vi "check Self Alignment Processing.vi"(8 "error in (no error)":errorcluster, 11 "Keysight 9020A in":refnum<class "Keysight 9020A.lvclass">) -> (0 "error out":errorcluster, 2 "On Alignment Processing":bool, 3 "Keysight 9020A out":refnum<class "Keysight 9020A.lvclass">)   [LabVIEW 2023, in "Spectrum Analyzer.lvlib" / "Keysight 9020A.lvclass"]
uses:
  Keysight 9020A.lvclass
  Keysight 9020A.lvclass/Keysight 9020A.ctl
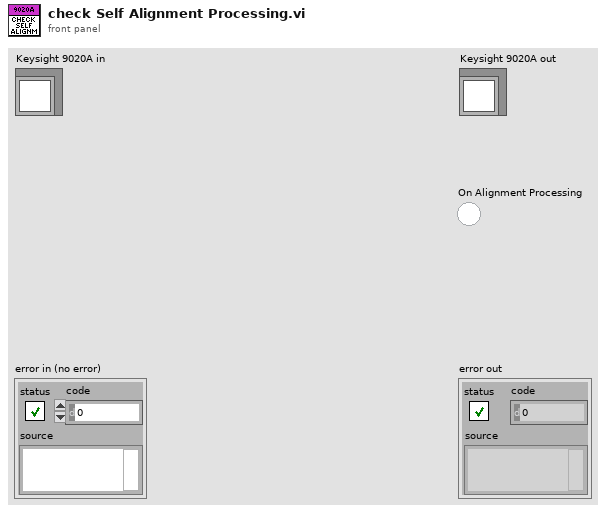
[diagram p1: front panel]
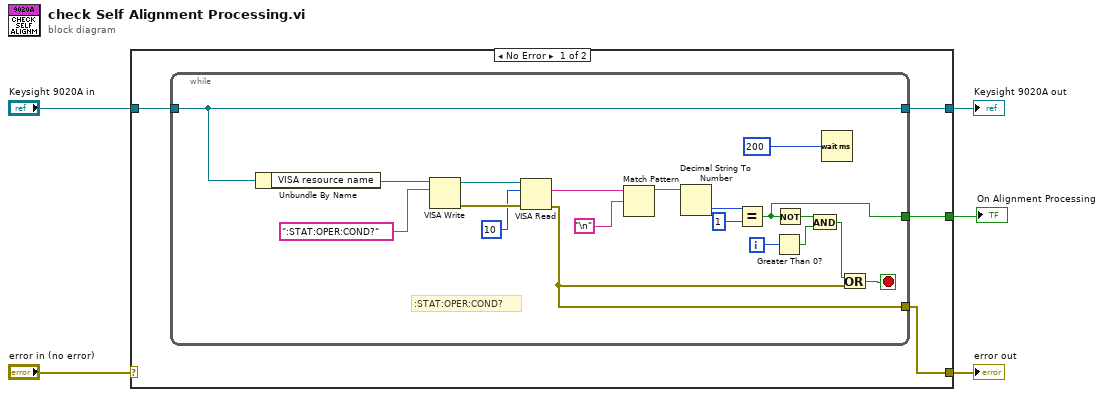
[diagram p0: block diagram]
diagram:
  n1 = case shown="No Error" "error in (no error)" {
    selector: "error in (no error)" -> [_ w30]
    tunnel: [w7 w30] -> w4
    tunnel: [w6 w29] -> w2
    tunnel: "Keysight 9020A in" -> [w9 w29]
    tunnel: [w8 _] -> w1
    frame No Error {
      n2 = while {
        tunnel: w9 -> [w16]
        tunnel: [w11] -> w8
        tunnel: [w17] -> w7
        tunnel: [w16] -> w6
        i -> [w12]
        stop <- w18 stop-if-true
        # ":STAT:OPER:COND?"
        n3 = Unbundle By Name(w16) -> ("VISA resource name"=w28:refnum<visa-resource-name>)
        n4 = VISA Write(VISA resource name=w28, write buffer=":STAT:OPER:COND?") -> (VISA resource name out=w26:refnum<visa-resource-name>, error out=w25:errorcluster)  [unwired: 1 in, 1 out]
        n5 = VISA Read(VISA resource name=w26, byte count=u32 10, error in (no error)=w25) -> (read buffer=w23:string, error out=w17:errorcluster)  [unwired: 2 out]
        n6 = Match Pattern(string=w23, regular expression="\n") -> (before substring=w21:string)  [unwired: 1 in, 3 out]
        n7 = Decimal String To Number(string=w21) -> (number=w20:i32)  [unwired: 2 in, 1 out]
        n8 = Equal?(x=w20, y=1) -> (x = y?=w11:bool)
        n9 = Greater Than 0?(x=w12) -> (x > 0?=w13:bool)
        n10 = Not(x=w11) -> (.not. x?=w14:bool)
        n11 = And(x=w14, y=w13) -> (x .and. y?=w10:bool)
        n12 = Wait (ms)(milliseconds to wait=u32 200) -> ()  [unwired: 1 out]
        n13 = Or(x=w10, y=w17) -> (x .or. y?=w18:bool)
      }
    }
    frame Error {
    }
  }
  "error out" <- w4
  "Keysight 9020A out" <- w2
  "On Alignment Processing" <- w1
